vi "Test Withdraw Funds Fast Cash 100.vi"() -> ()   [LabVIEW 2026]
doc: "Caraya unit test for Withdraw Funds.vi with the amount of the Fast Cash $100 menu item (feature #47). The Fast Cash $100 state of the main VI calls Withdraw Funds.vi with Amount 100, exactly as Fast Cash $50 does with 50.\n\nEvery case starts from its own fresh copy of the specification accounts file (Create Accounts Fixture.vi, written under Tests\\results), so the real ATM accounts.txt is never touched and the cases can run in parallel. The balance is always checked by reading the file back with Get Account.vi. The expected records are instances of the typedef ATM Account.ctl.\n\nCase 1: withdrawing 100 from 23456 (balance 1000) succeeds and the file holds 900.\nCase 2: account 12345 (balance 550) is first brought down to 50 by withdrawing 500, the set-up step. Withdrawing 100 is then refused (Sufficient Funds? FALSE) and the file still holds 50 - the Withdrawal Failed path.\n\nThe error cluster carries the FIRST failure only. Read the JUnit report for all of them."
uses:
  Controls/ATM Account.ctl
  <vilib>/addons/_JKI Toolkits/Caraya/classes/Test/Test.lvclass
  <vilib>/addons/_JKI Toolkits/Caraya/classes/Assert/Assert.lvclass
panel:
  out "error out":errorcluster
  in  "error in":errorcluster
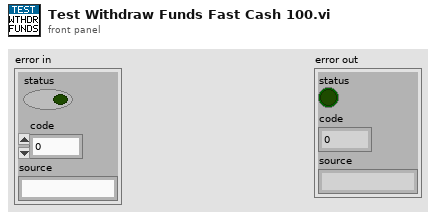
[diagram p1: front panel]
types:
  T1 = typedef "ATM Account.ctl" = cluster{"Account Number":string, "First Name":string, "Last Name":string, "Balance":dbl}
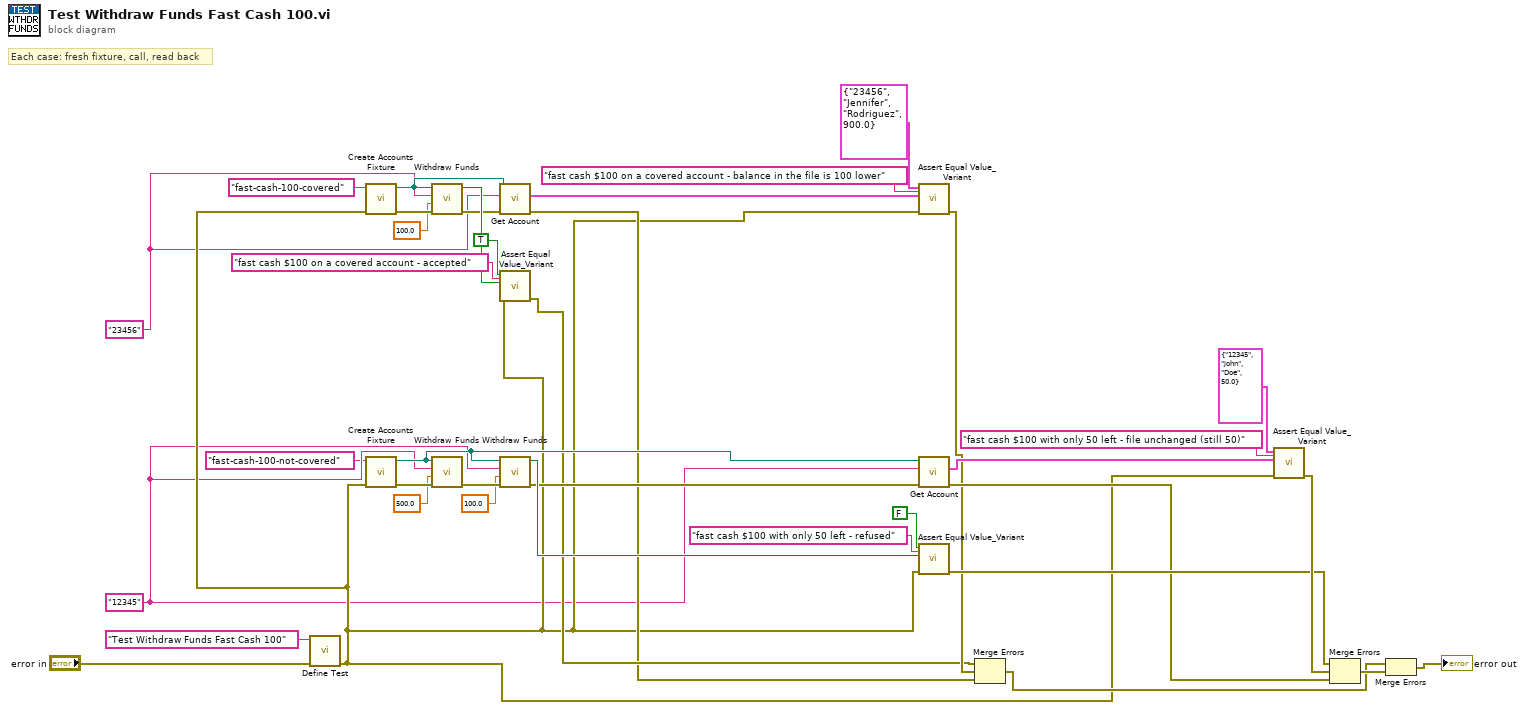
[diagram p0: block diagram]
diagram:
  w12 = "12345" ("Account Number 2")
  w5 = "23456" ("Account Number 1")
  # "Each case: fresh fixture, call, read back"
  n1 = call <vilib>:"Define Test.vi"("error in (no error)"="error in", "Label (VI Title)"="Test Withdraw Funds Fast Cash 100") -> ("error out"=w19:errorcluster)  [unwired: 8 in, 1 out]
  n2 = call "Create Accounts Fixture.vi"("error in"=w19, "Fixture Name"="fast-cash-100-covered" ("Fixture Name 1")) -> ("error out"=w20:errorcluster, "Accounts File Path"=w21:path)  [unwired: 8 in]
  n3 = call "Create Accounts Fixture.vi"("error in"=w19, "Fixture Name"="fast-cash-100-not-covered" ("Fixture Name 2")) -> ("error out"=w28:errorcluster, "Accounts File Path"=w29:path)  [unwired: 8 in]
  n4 = call "Withdraw Funds.vi"("error in"=w20, "Amount"=100.0 ("Amount 1"), "Account Number"=w5, "Accounts File Path"=w21) -> ("error out"=w22:errorcluster, "Sufficient Funds?"=w23:bool)  [unwired: 5 in, 1 out]
  n5 = call "Withdraw Funds.vi"("error in"=w28, "Amount"=500.0 ("Setup Amount 2"), "Account Number"=w12, "Accounts File Path"=w29) -> ("error out"=w30:errorcluster)  [unwired: 5 in, 2 out]
  n6 = call "Get Account.vi"("error in"=w22, "Account Number"=w5, "Accounts File Path"=w21) -> ("error out"=w24:errorcluster, "Account"=w25:T1)  [unwired: 6 in, 1 out]
  n7 = call <vilib>:"Assert Equal Value_Variant.vi"("Label"="fast cash $100 on a covered account - accepted" ("Label 1"), "error in (no error)"=w19, "Actual"=w23, "Expected"=TRUE ("expected 1")) -> ("error out"=w26:errorcluster)  [unwired: 6 in, 1 out]
  n8 = call "Withdraw Funds.vi"("error in"=w30, "Amount"=100.0 ("Amount 2"), "Account Number"=w12, "Accounts File Path"=w29) -> ("error out"=w31:errorcluster, "Sufficient Funds?"=w32:bool)  [unwired: 5 in, 1 out]
  n9 = call <vilib>:"Assert Equal Value_Variant.vi"("Label"="fast cash $100 on a covered account - balance in the file is 100 lower" ("Label 2"), "error in (no error)"=w19, "Actual"=w25, "Expected"=T1 {"Account Number"="23456", "First Name"="Jennifer", "Last Name"="Rodriguez", "Balance"=900.0} ("expected 2")) -> ("error out"=w27:errorcluster)  [unwired: 6 in, 1 out]
  n10 = call "Get Account.vi"("error in"=w31, "Account Number"=w12, "Accounts File Path"=w29) -> ("error out"=w33:errorcluster, "Account"=w34:T1)  [unwired: 6 in, 1 out]
  n11 = call <vilib>:"Assert Equal Value_Variant.vi"("Label"="fast cash $100 with only 50 left - refused" ("Label 3"), "error in (no error)"=w19, "Actual"=w32, "Expected"=FALSE ("expected 3")) -> ("error out"=w35:errorcluster)  [unwired: 6 in, 1 out]
  n12 = Merge Errors(w26, w27, w24) -> (w37:errorcluster)
  n13 = call <vilib>:"Assert Equal Value_Variant.vi"("Label"="fast cash $100 with only 50 left - file unchanged (still 50)" ("Label 4"), "error in (no error)"=w19, "Actual"=w34, "Expected"=T1 {"Account Number"="12345", "First Name"="John", "Last Name"="Doe", "Balance"=50.0} ("expected 4")) -> ("error out"=w36:errorcluster)  [unwired: 6 in, 1 out]
  n14 = Merge Errors(w35, w36, w33) -> (w38:errorcluster)
  n15 = Merge Errors(w37, w38) -> (→"error out":errorcluster)
